vi "[ex ce] Calc Spectrum.vi"() -> ()   [LabVIEW 2021]
doc: "<B>Signal processing example</B>\n\nA script in this example generates a compound signal and computes power spectrum of it.\n\nInput parameters for computation are passed from controls on the VI Front Panel. Results are displayed in the VI indicators.\n\n<B>Remark</B>\nSome functions in this example use VIs of Advanced Analysis Package. The example doesn't work properly if you don't have these VIs.\n\n::: CalcExpress Toolkit :::\nCopyright (c) 2000-2026 Konstantin Shifershteyn. All rights reserved."
panel:
  in  "F2":dbl(slide)=121.0 min=0.0 max=200.0 step=1.0 scale=0.0..200.0
  in  "F1":dbl(slide)=51.0 min=10.0 max=200.0 step=1.0 scale=0.0..200.0
  in  "ANoise":dbl(slide) scale=0.0..100.0
  in  "A2":dbl(slide)=36.708860759493675 scale=0.0..100.0
  in  "A1":dbl(slide)=50.63291139240506 scale=0.0..100.0
  in  "Spectrum frequency interval - Variable Name":string="df"
  in  "Spectrum magnitude - Variable Name":string="Spectrum"
  out "spectrum":cluster{dbl, "value out":dbl, "value out":dbl[]}(graph)
  in  "Input Waveform - Variable Name":string="Signal"
  out "WaveForm":dbl[](graph)
  in  "stop":bool
  in  "Expression":string="/* variables definition */\ndbl(\"Ph1\",0); dbl(\"Ph2\",0); dbl(\"df\");\na1dbl(\"Signal\"); a1dbl(\"Sig1\"); a1dbl(\"Sig2\");\na1dbl(\"Spectrum\");\n\nFs=1000; // Sampling frequency\nNs=100;  // Number of samples\n\n/* Create Signal from two waveforms */\nPh1 = SineWave(Sig1, Ns, F1/Fs, A1, Ph1);\nPh2 = SineWave(Sig2, Ns, F2/Fs, A2, Ph2);\nSignal = Sig1 + Sig2;\n\n/* add uniform white noise to Signal */\nSignal += UWNoise(Ns, ANoise);\n\n/* compute the power spectrum */\ndf = APSpectrum(Signal, Spectrum, 1/Fs);"
  # "Frequency (values for the respective variables)"
  # "Amplitude (values for the respective variables)"
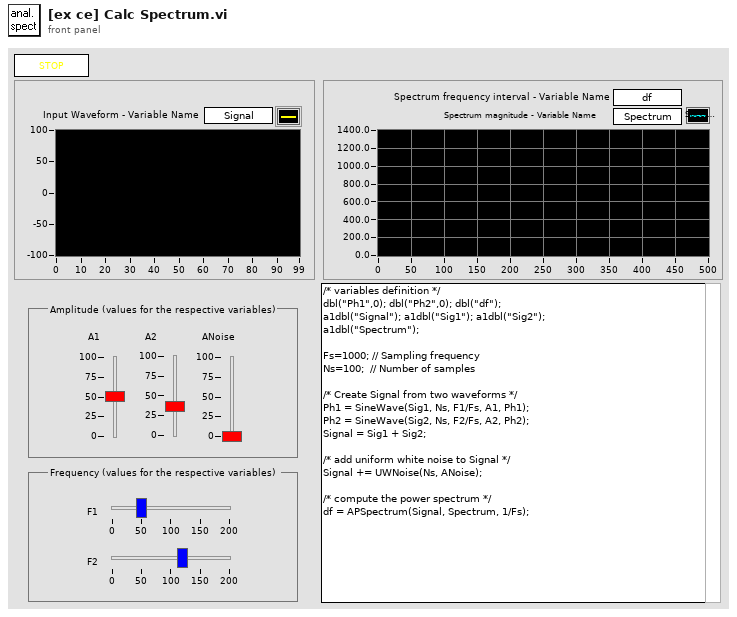
[diagram p1: front panel]
types:
  T1 = enum32{"nothing", "reset", "assign name", "get name", "get handle"}
  T2 = typedef "VarMan Variable Context Handle.ctl" = i32
  T3 = enum16{"create", "destroy", "set value", "get value"}
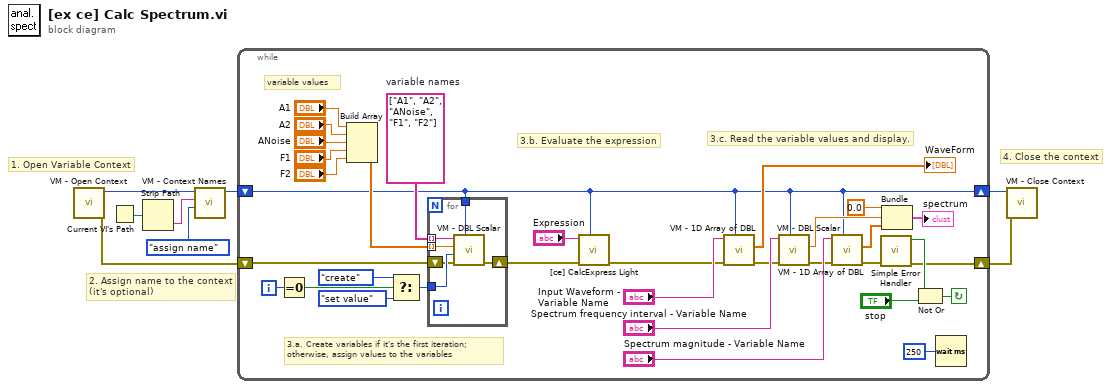
[diagram p0: block diagram]
diagram:
  # "4. Close the context"
  # "1. Open Variable Context"
  # "2. Assign name to the context\n(it's optional)"
  n1 = call "VM - Open Context.vi"() -> ("error out"=w4:errorcluster, "VC Handle out"=w2:T2)  [unwired: 9 in, 1 out]
  n2 = Current VI's Path() -> (path=w6:path)
  n3 = Strip Path(path=w6) -> (name=w5:string)  [unwired: 1 out]
  n4 = call "VM - Context Names.vi"("action"=T1."assign name", "VC Name"=w5, "VC Handle"=w2) -> ("VC Handle out"=w3:T2)  [unwired: 3 in, 3 out]
  n5 = while {
    shift-left: w4 -> [w11]
    shift-right: [w10] -> w8
    shift-right: [w9] -> w1
    shift-left: w3 -> [w9]
    i -> [w13]
    stop <- w40 continue-if-true
    w16 = string[] ["A1", "A2", "ANoise", "F1", "F2"]  # variable names
    # "3.c. Read the variable values and display."
    # "3.b. Evaluate the expression"
    # "3.a. Create variables if it's the first iteration;\notherwise, assign values to the variables"
    # "variable values"
    n6 = Equal To 0?(x=w13) -> (x = 0?=w23:bool)
    n7 = Build Array("A1", "A2", "ANoise", "F1", "F2") -> (w20:dbl[])
    n8 = Select(t=T3."create" ("cmd"), s=w23, f=T3."set value" ("cmd")) -> (s? t:f=w24:T3)
    n9 = for {
      tunnel: w24 -> [w47]
      tunnel: w20 -> [w46] mode=indexing
      tunnel: w16 -> [w45] mode=indexing
      shift-right: [w44] -> w12
      shift-left: w11 -> [w43]
      tunnel: w9 -> [w42]
      n10 = call "VM - DBL Scalar.vi"("VC Handle"=w42, "error in"=w43, "cmd"=w47, "value in"=w46, "name_spec"=w45) -> ("error out"=w44:errorcluster)  [unwired: 1 in, 5 out]
    }
    n11 = call "[ce] CalcExpress Light.vi"("VC Handle"=w9, "error in"=w12, "expression"="Expression") -> ("error out"=w30:errorcluster)  [unwired: 6 in, 2 out]
    n12 = call "VM - 1D Array of DBL.vi"("VC Handle"=w9, "error in"=w30, "name_spec"="Input Waveform - Variable Name") -> ("error out"=w29:errorcluster, "value out"=→"WaveForm":dbl[])  [unwired: 3 in, 4 out]
    n13 = call "VM - DBL Scalar.vi"("VC Handle"=w9, "error in"=w29, "name_spec"="Spectrum frequency interval - Variable Name") -> ("error out"=w28:errorcluster, "value out"=w39:dbl)  [unwired: 3 in, 4 out]
    n14 = call "VM - 1D Array of DBL.vi"("VC Handle"=w9, "error in"=w28, "name_spec"="Spectrum magnitude - Variable Name") -> ("error out"=w27:errorcluster, "value out"=w36:dbl[])  [unwired: 3 in, 4 out]
    n15 = call <vilib>:"Simple Error Handler.vi"("error in (no error)"=w27) -> ("error?"=w25:bool, "error out"=w10:errorcluster)  [unwired: 4 in, 3 out]
    n16 = Bundle(0.0, "value out"=w39, "value out"=w36) -> (→"spectrum":cluster{dbl, "value out":dbl, "value out":dbl[]})  [unwired: 1 in]
    n17 = Not Or(1:"stop", 2:w25) -> (0:w40:bool)
    n18 = Wait (ms)(milliseconds to wait=u32 250) -> ()  [unwired: 1 out]
  }
  n19 = call "VM - Close Context.vi"("error in"=w8, "VC Handle"=w1) -> ()  [unwired: 8 in, 2 out]
